vi "Configure Control.vi"(8 "error in (no error)":errorcluster, 10 "control":refnum<vi>, 11 "NT Scalar (Numeric) in":refnum<class "NT Scalar (Numeric).lvclass">) -> (0 "error out":errorcluster, 2 "control out":refnum<vi>, 3 "NT Scalar (Numeric) out":refnum<class "NT Scalar (Numeric).lvclass">)   [LabVIEW 2020, in "PV Access.lvlib" / "PV Data.lvlib" / "NT Scalar (Numeric).lvclass"]
doc: "Set the description of <B>control</B> from the value's metadata."
uses:
  NT Scalar (Numeric).lvclass
  NT Scalar/NT Scalar.lvclass
  NT Scalar (Numeric).lvclass/NT Scalar (Numeric).ctl
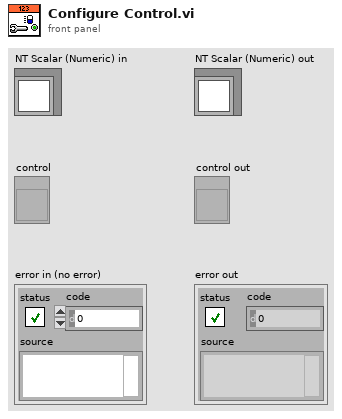
[diagram p1: front panel]
types:
  T1 = typedef "PV Access.lvlib/PV Data.lvlib/Display Form.ctl" = enum16{"Default", "String", "Binary", "Decimal", "Hex", "Exponential", "Engineering"}
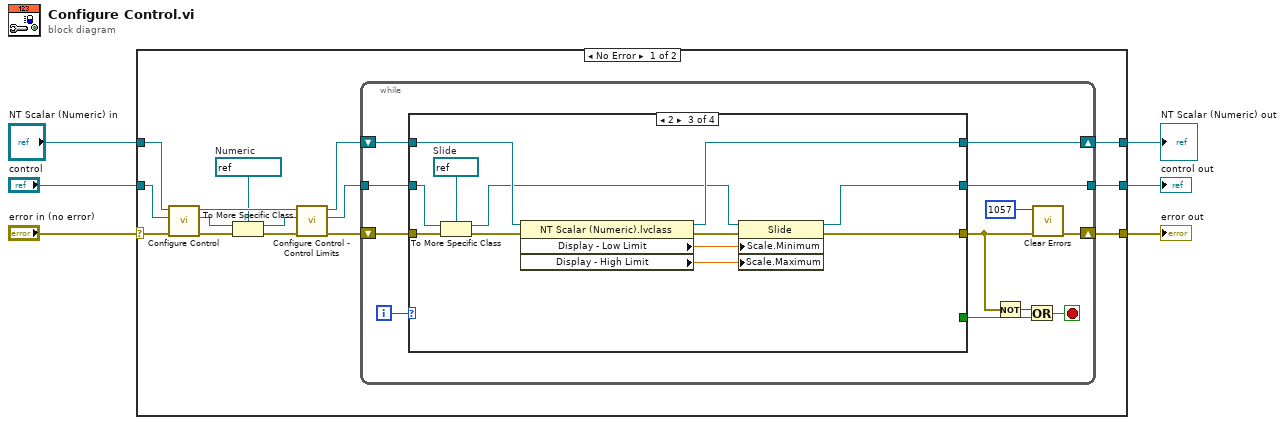
[diagram p0: block diagram]
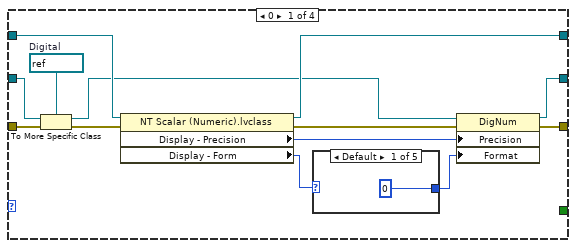
[diagram p2: hidden frame]
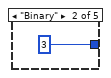
[diagram p3: hidden frame]
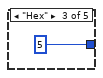
[diagram p4: hidden frame]
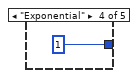
[diagram p5: hidden frame]
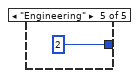
[diagram p6: hidden frame]
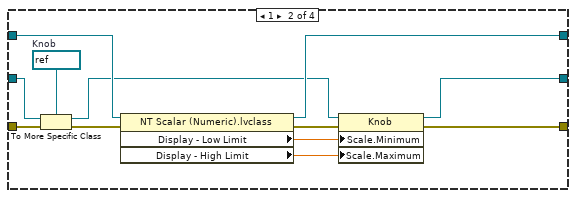
[diagram p7: hidden frame]
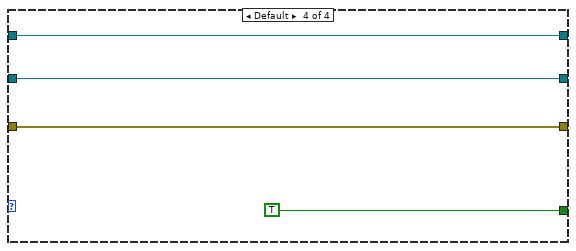
[diagram p8: hidden frame]
diagram:
  n1 = case shown="No Error" "error in (no error)" {
    selector: "error in (no error)" -> [w21 w80]
    tunnel: [w7 w80] -> w6
    tunnel: "control" -> [w19 w81]
    tunnel: "NT Scalar (Numeric) in" -> [w17 w82]
    tunnel: [w11 w82] -> w2
    tunnel: [w8 w81] -> w1
    frame No Error {
      w15 = refnum<vi> refnum  # Numeric
      n2 = call-parent "Configure Control.vi"("error in (no error)"=w21, "control"=w19, "Base in"=w17) -> ("error out"=w20:errorcluster, "control out"=w18:refnum<vi>, "Base out"=w16:refnum<class "NT Scalar (Numeric).lvclass">)  [unwired: 6 in]
      n3 = To More Specific Class(target class=w15, reference=w18, error in=w20) -> (specific class reference=w13:refnum<vi>, error out=w14:errorcluster)
      n4 = call-dynamic "Configure Control - Control Limits.vi"("error in (no error)"=w14, "control in"=w13, "Has Control Limits in"=w16) -> ("error out"=w10:errorcluster, "control out"=w9:refnum<vi>, "Has Control Limits out"=w12:refnum<class "NT Scalar (Numeric).lvclass">)  [unwired: 6 in]
      n5 = while {
        shift-right: [w32] -> w11
        shift-left: w12 -> [w33]
        shift-right: [w22] -> w7
        shift-left: w10 -> [w31]
        tunnel: w9 -> [w30]
        tunnel: [w29] -> w8
        i -> [w28]
        stop <- w26 stop-if-true
        n6 = case shown="2" w28 {
          tunnel: w33 -> [w42 w57 w69 w78]
          tunnel: [w41 w56 w68 w78] -> w32
          tunnel: w30 -> [w35 w61 w73 w77]
          tunnel: [w40 w58 w70 w79] -> w23
          tunnel: [w39 w52 w64 w77] -> w29
          tunnel: w31 -> [w37 w62 w74 w79]
          tunnel: [_ _ _ TRUE] -> w25
          frame 0 {
            w38 = refnum<vi> refnum  # Digital
            n7 = To More Specific Class(target class=w38, reference=w35, error in=w37) -> (specific class reference=w34:refnum<vi>, error out=w36:errorcluster)
            n8 = property class="NT Scalar (Numeric).lvclass"(reference=w42, error in=w36) -> (reference out=w41:refnum<class "NT Scalar (Numeric).lvclass">, error out=w45:errorcluster, "Display - Precision"=w44:i32, "Display - Form"=w43:T1)
            n9 = case shown="Default" w43 {
              tunnel: [u8 0 u8 3 u8 5 u8 1 u8 2] -> w46
              frame Default {
              }
              frame "Binary" {
              }
              frame "Hex" {
              }
              frame "Exponential" {
              }
              frame "Engineering" {
              }
            }
            n10 = property on="Property Node" class="DigNum"(reference=w34, error in=w45, "Precision"=w44, "Format"=w46) -> (reference out=w39:refnum<vi>, error out=w40:errorcluster)
          }
          frame 1 {
            w63 = refnum<vi> refnum  # Knob
            n11 = To More Specific Class(target class=w63, reference=w61, error in=w62) -> (specific class reference=w55:refnum<vi>, error out=w60:errorcluster)
            n12 = property class="NT Scalar (Numeric).lvclass"(reference=w57, error in=w60) -> (reference out=w56:refnum<class "NT Scalar (Numeric).lvclass">, error out=w59:errorcluster, "Display - Low Limit"=w54:dbl, "Display - High Limit"=w53:dbl)
            n13 = property on="Property Node" class="Knob"(reference=w55, error in=w59, "Scale.Minimum"=w54, "Scale.Maximum"=w53) -> (reference out=w52:refnum<vi>, error out=w58:errorcluster)
          }
          frame 2 {
            w75 = refnum<vi> refnum  # Slide
            n14 = To More Specific Class(target class=w75, reference=w73, error in=w74) -> (specific class reference=w67:refnum<vi>, error out=w72:errorcluster)
            n15 = property class="NT Scalar (Numeric).lvclass"(reference=w69, error in=w72) -> (reference out=w68:refnum<class "NT Scalar (Numeric).lvclass">, error out=w71:errorcluster, "Display - Low Limit"=w66:dbl, "Display - High Limit"=w65:dbl)
            n16 = property on="Property Node" class="Slide"(reference=w67, error in=w71, "Scale.Minimum"=w66, "Scale.Maximum"=w65) -> (reference out=w64:refnum<vi>, error out=w70:errorcluster)
          }
          frame Default {
          }
        }
        n17 = Not(x=w23) -> (.not. x?=w27:bool)
        n18 = Or(x=w27, y=w25) -> (x .or. y?=w26:bool)
        n19 = call <vilib>:"Clear Errors.vi"("error in (no error)"=w23, "specific error code to clear (0: all)"=1057) -> ("error out"=w22:errorcluster)  [unwired: 4 in, 1 out]
      }
    }
    frame Error {
    }
  }
  "error out" <- w6
  "NT Scalar (Numeric) out" <- w2
  "control out" <- w1
